vi "Receive Messages.vi"(6 "Wait Time":i32=-1, 8 "error in (no error)":errorcluster, 9 "Visibility Timeout":i32, 10 "Max Number of Messages":i32=1, 11 "SQS in":refnum<class "Queue.lvclass">) -> (0 "error out":errorcluster, 2 "Messages":T1[](array[typedef]), 3 "SQS out":refnum<class "Queue.lvclass">)   [LabVIEW 2015, in "NI_AWS_SQS.lvlib" / "Queue.lvclass"]
doc: "Retrieves one or more messages (up to 10), from the specified queue. Using the Wait Time parameter enables long-poll support. For more information, see Amazon SQS Long Polling in the Amazon SQS Developer Guide.\n\nShort poll is the default behavior where a weighted random set of machines is sampled on a ReceiveMessage call. Thus, only the messages on the sampled machines are returned. If the number of messages in the queue is small (fewer than 1,000), you most likely get fewer messages than you requested per ReceiveMessage call. If the number of messages in the queue is extremely small, you might not receive any messages in a particular ReceiveMessage response. If this happens, repeat the request.\n\nFor each message returned, the response includes the following:\n\nThe message body.\nAn MD5 digest of the message body. For information on MD5, see RFC1321.\nThe MessageId you received when you sent the message to the queue.\nThe receipt handle.\nThe message attributes.\nAn MD5 digest of the message attributes.\nThe receipt handle is the identifier you must provide when deleting the message. For more information, see Queue and Message Identifiers in the Amazon SQS Developer Guide.\n\nYou can provide the VisibilityTimeout parameter in your request. The parameter is applied to the messages that Amazon SQS returns in the response. If you don't include the parameter, the overall visibility timeout for the queue is used for the returned messages. For more information, see Visibility Timeout in the Amazon SQS Developer Guide.\n\nA message that isn't deleted or a message whose visibility isn't extended before the visibility timeout expires counts as a failed receive. Depending on the configuration of the queue, the message might be sent to the dead letter queue.\n\nNote\nIn the future, new attributes might be added. If you write code that calls this action, we recommend that you structure your code so that it can handle new attributes gracefully."
uses:
  Queue.lvclass
  Message.ctl
  Message Attribute Value Pair.ctl
  Message Attribute.ctl
  Custom Attribute.ctl
  Custom Attribute Type.ctl
  Core/HTTP Request/Name Value Pair.ctl
  Core/HTTP Request/Request Options.ctl
  Core/HTTP Request/Region handling.ctl
  Core/HTTP Request/URL formatting.ctl
  Queue.lvclass/Queue.ctl
  Read Account Number.vi
  Read Name.vi
  Core/HTTP Request/HTTP Request.lvclass
  XML Parsing/NI_XML Parsing.lvlib
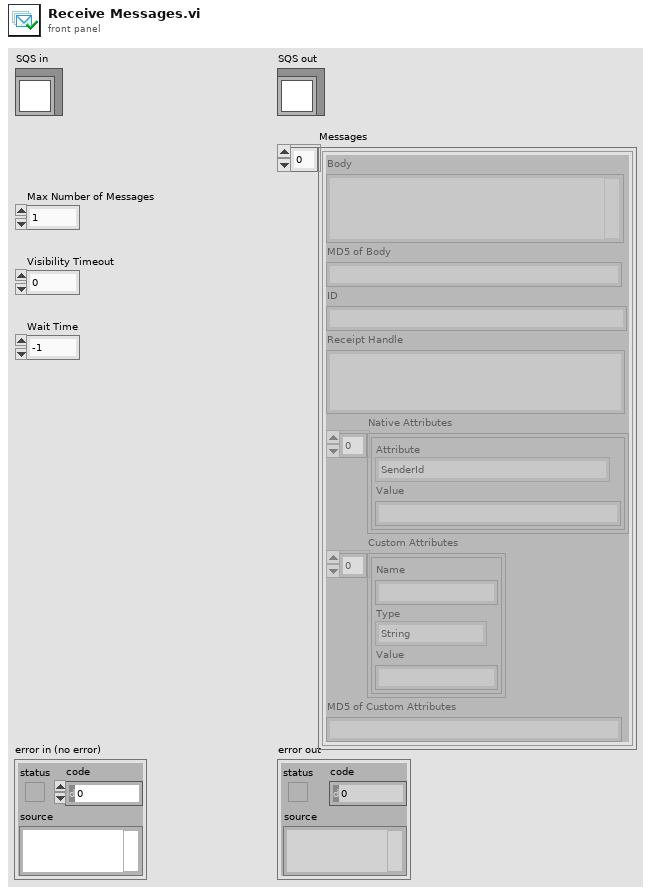
[diagram p1: front panel]
types:
  T1 = typedef "NI_AWS_SQS.lvlib/Queue.lvclass/Message.ctl" = cluster{"Body":string, "MD5 of Body":string, "ID":string, "Receipt Handle":string, "Native Attributes":T2[], "Custom Attributes":T4[], "MD5 of Custom Attributes":string}
  T2 = typedef "NI_AWS_SQS.lvlib/Queue.lvclass/Message Attribute Value Pair.ctl" = cluster{"Attribute":T3, "Value":string}
  T3 = typedef "NI_AWS_SQS.lvlib/Queue.lvclass/Message Attribute.ctl" = enum16{"SenderId", "SentTimestamp", "ApproximateReceiveCount", "ApproximateFirstReceiveTimestamp"}
  T4 = typedef "NI_AWS_SQS.lvlib/Queue.lvclass/Custom Attribute.ctl" = cluster{"Name":string, "Type":T5, "Value":string}
  T5 = typedef "NI_AWS_SQS.lvlib/Queue.lvclass/Custom Attribute Type.ctl" = enum16{"String", "Number", "Binary"}
  T6 = typedef "NI_AWS_Core.lvlib/HTTP Request.lvclass/Name Value Pair.ctl" = cluster{"name":string, "value":string}
  T7 = typedef "NI_AWS_Core.lvlib/HTTP Request.lvclass/Request Options.ctl" = cluster{"request headers":T6[], "request parameters":T6[], "request body":string, "region handling":T8, "URL formatting":T9}
  T8 = typedef "NI_AWS_Core.lvlib/HTTP Request.lvclass/Region handling.ctl" = enum16{"use region everywhere", "use region (authentication only)", "use region (URL only)", "ignore region everwhere"}
  T9 = typedef "NI_AWS_Core.lvlib/HTTP Request.lvclass/URL formatting.ctl" = enum16{"region-", "region."}
  T10 = typedef "NI_AWS_Core.lvlib/HTTP Request.lvclass/Response.ctl" = cluster{"Headers":string, "Body":string}
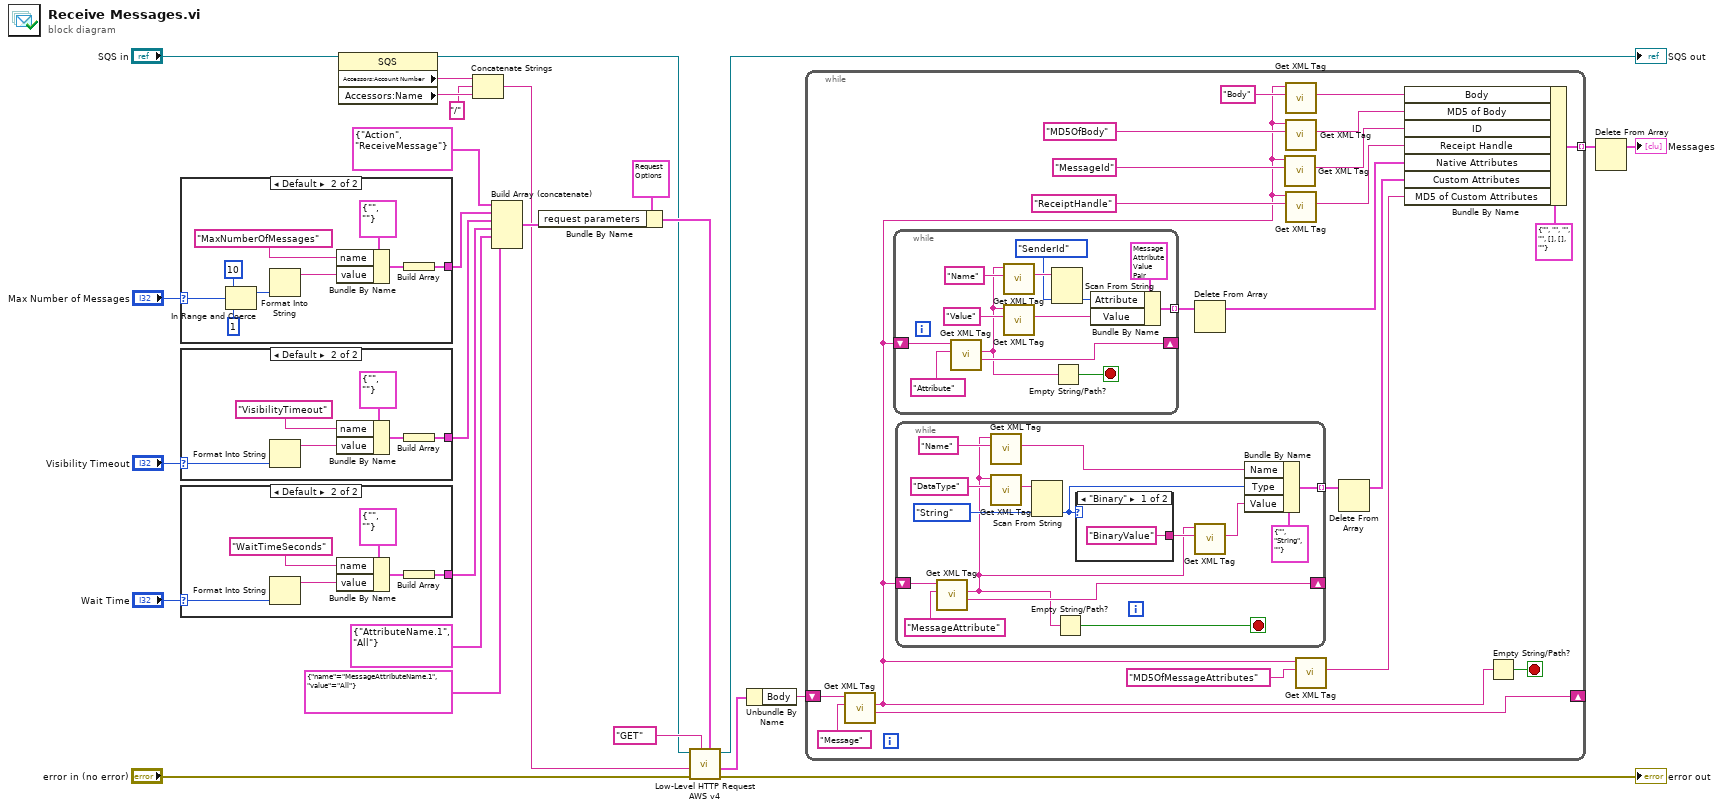
[diagram p0: block diagram]
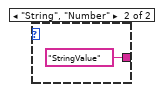
[diagram p2: hidden frame]
diagram:
  n1 = case shown="Default" "Max Number of Messages" {
    selector: "Max Number of Messages" -> [_ w33]
    tunnel: [_ w27] -> w15
    frame ..1 {
    }
    frame Default {
      n2 = In Range and Coerce(upper limit=10, x=w33, lower limit=1) -> (coerced(x)=w30:i32)  [unwired: 1 out]
      n3 = Format Into String(w30) -> (resulting string=w29:string)  [unwired: 3 in, 1 out]
      n4 = Bundle By Name(cluster=T6 {"name"="", "value"=""} ("element"), "name"="MaxNumberOfMessages", "value"=w29) -> (w28:T6)
      n5 = Build Array(w28) -> (w27:T6[])
    }
  }
  n6 = case shown="Default" "Visibility Timeout" {
    selector: "Visibility Timeout" -> [_ w41]
    tunnel: [_ w36] -> w13
    frame ..0 {
    }
    frame Default {
      n7 = Format Into String(w41) -> (resulting string=w38:string)  [unwired: 3 in, 1 out]
      n8 = Bundle By Name(cluster=T6 {"name"="", "value"=""} ("element"), "name"="VisibilityTimeout", "value"=w38) -> (w37:T6)
      n9 = Build Array(w37) -> (w36:T6[])
    }
  }
  n10 = case shown="Default" "Wait Time" {
    selector: "Wait Time" -> [_ w47]
    tunnel: [_ w42] -> w11
    frame ..-1 {
    }
    frame Default {
      n11 = Format Into String(w47) -> (resulting string=w44:string)  [unwired: 3 in, 1 out]
      n12 = Bundle By Name(cluster=T6 {"name"="", "value"=""} ("element"), "name"="WaitTimeSeconds", "value"=w44) -> (w43:T6)
      n13 = Build Array(w43) -> (w42:T6[])
    }
  }
  n14 = property class="SQS"(reference="SQS in") -> (reference out=w2:refnum<class "Queue.lvclass">, "Accessors:Account Number"=w21:string, "Accessors:Name"=w20:string)  [unwired: 1 in, 1 out]
  n15 = Concatenate Strings(w21, "/", w20) -> (w18:string)
  n16 = Build Array (concatenate)(T6 {"name"="Action", "value"="ReceiveMessage"} ("Cluster"), w15, w13, w11, T6 {"name"="AttributeName.1", "value"="All"} ("Cluster"), T6 {"name"="MessageAttributeName.1", "value"="All"} ("Cluster")) -> (w22:T6[])
  n17 = Bundle By Name(cluster=T7 {"request headers"=[], "request parameters"=[{"name"="Action", "value"="ListQueues"}], "request body"="", "region handling"=enum."use region everywhere", "URL formatting"=enum."region."} ("Request Options"), "request parameters"=w22) -> (w3:T7)
  n18 = call "Low-Level HTTP Request AWS v4.vi"("Request Options"=w3, "HTTP-Verb"="GET", "error in (no error)"="error in (no error)", "URL Suffix"=w18, "AWS Core in"=w2) -> ("error out"=→"error out":errorcluster, "Response"=w5:T10, "AWS Core out"=→"SQS out":refnum<class "Queue.lvclass">)  [unwired: 3 in, 1 out]
  n19 = Unbundle By Name(w5) -> ("Body"=w24:string)
  n20 = while {
    shift-right: [w67] -> _
    shift-left: w24 -> [w68]
    tunnel: [w62] -> w9 mode=indexing
    stop <- w66 stop-if-true
    n21 = call "Get XML Tag.vi"("Tag name"="Message", "XML String in"=w68) -> ("Remaining string"=w67:string, "Tag value"=w50:string)  [unwired: 5 in, 3 out]
    n22 = while {
      shift-right: [w80] -> _
      shift-left: w50 -> [w81]
      tunnel: [w76] -> w54 mode=indexing
      stop <- w78 stop-if-true
      n23 = call "Get XML Tag.vi"("Tag name"="Attribute", "XML String in"=w81) -> ("Remaining string"=w80:string, "Tag value"=w73:string)  [unwired: 5 in, 3 out]
      n24 = call "Get XML Tag.vi"("Tag name"="Name", "XML String in"=w73) -> ("Tag value"=w70:string)  [unwired: 5 in, 4 out]
      n25 = call "Get XML Tag.vi"("Tag name"="Value", "XML String in"=w73) -> ("Tag value"=w72:string)  [unwired: 5 in, 4 out]
      n26 = Scan From String(input string=w70, default 1=Message_Attribute."SenderId" ("Attribute")) -> (output 1=w71:T3)  [unwired: 3 in, 3 out]
      n27 = Empty String/Path?(string/path=w73) -> (empty?=w78:bool)
      n28 = Bundle By Name(cluster=T2 {"Attribute"=enum."ApproximateFirstReceiveTimestamp", "Value"=""} ("Message Attribute Value Pair"), "Attribute"=w71, "Value"=w72) -> (w76:T2)
    }
    n29 = while {
      shift-right: [w95] -> _
      shift-left: w50 -> [w96]
      tunnel: [w92] -> w52 mode=indexing
      stop <- w93 stop-if-true
      n30 = call "Get XML Tag.vi"("Tag name"="MessageAttribute", "XML String in"=w96) -> ("Remaining string"=w95:string, "Tag value"=w82:string)  [unwired: 5 in, 3 out]
      n31 = call "Get XML Tag.vi"("Tag name"="Name", "XML String in"=w82) -> ("Tag value"=w88:string)  [unwired: 5 in, 4 out]
      n32 = call "Get XML Tag.vi"("Tag name"="DataType", "XML String in"=w82) -> ("Tag value"=w87:string)  [unwired: 5 in, 4 out]
      n33 = Scan From String(input string=w87, default 1=Custom_Attribute_Type."String" ("Custom Attribute Type")) -> (output 1=w85:T5)  [unwired: 3 in, 3 out]
      n34 = Empty String/Path?(string/path=w82) -> (empty?=w93:bool)
      n35 = case shown="\"Binary\"" w85 {
        tunnel: ["BinaryValue" "StringValue"] -> w84
        frame "Binary" {
        }
        frame "String", "Number" {
        }
      }
      n36 = call "Get XML Tag.vi"("Tag name"=w84, "XML String in"=w82) -> ("Tag value"=w83:string)  [unwired: 5 in, 4 out]
      n37 = Bundle By Name(cluster=T4 {"Name"="", "Type"=enum."String", "Value"=""} ("Custom Attribute"), "Name"=w88, "Type"=w85, "Value"=w83) -> (w92:T4)
    }
    n38 = Delete From Array(array=w54) -> (array with subset deleted=w53:T2[])  [unwired: 2 in, 1 out]
    n39 = call "Get XML Tag.vi"("Tag name"="MessageId", "XML String in"=w50) -> ("Tag value"=w58:string)  [unwired: 5 in, 4 out]
    n40 = call "Get XML Tag.vi"("Tag name"="Body", "XML String in"=w50) -> ("Tag value"=w59:string)  [unwired: 5 in, 4 out]
    n41 = call "Get XML Tag.vi"("Tag name"="MD5OfBody", "XML String in"=w50) -> ("Tag value"=w61:string)  [unwired: 5 in, 4 out]
    n42 = call "Get XML Tag.vi"("Tag name"="ReceiptHandle", "XML String in"=w50) -> ("Tag value"=w55:string)  [unwired: 5 in, 4 out]
    n43 = call "Get XML Tag.vi"("Tag name"="MD5OfMessageAttributes", "XML String in"=w50) -> ("Tag value"=w49:string)  [unwired: 5 in, 4 out]
    n44 = Delete From Array(array=w52) -> (array with subset deleted=w51:T4[])  [unwired: 2 in, 1 out]
    n45 = Bundle By Name(cluster=T1 {"Body"="", "MD5 of Body"="", "ID"="", "Receipt Handle"="", "Native Attributes"=[], "Custom Attributes"=[], "MD5 of Custom Attributes"=""} ("Message"), "Body"=w59, "MD5 of Body"=w61, "ID"=w58, "Receipt Handle"=w55, "Native Attributes"=w53, "Custom Attributes"=w51, "MD5 of Custom Attributes"=w49) -> (w62:T1)
    n46 = Empty String/Path?(string/path=w50) -> (empty?=w66:bool)
  }
  n47 = Delete From Array(array=w9) -> (array with subset deleted=→"Messages":T1[])  [unwired: 2 in, 1 out]
